vi "ALL - FuncVIs Collection.vi"() -> ()   [LabVIEW 2021]
doc: "::: CalcExpress Toolkit :::\nCopyright (c) 2000-2026 Konstantin Shifershteyn. All rights reserved."
uses:
  cetypes.llb/CalcExpress Instance RefNum.ctl
panel:
  in  "False":bool
  in  "InstanceRef":T1
  # "CalcExpress Toolkit\n\nFuncVI Collection"
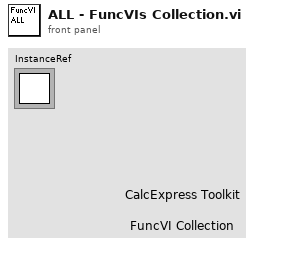
[diagram p1: front panel]
types:
  T1 = typedef "CalcExpress Instance RefNum.ctl" = refnum<k1>
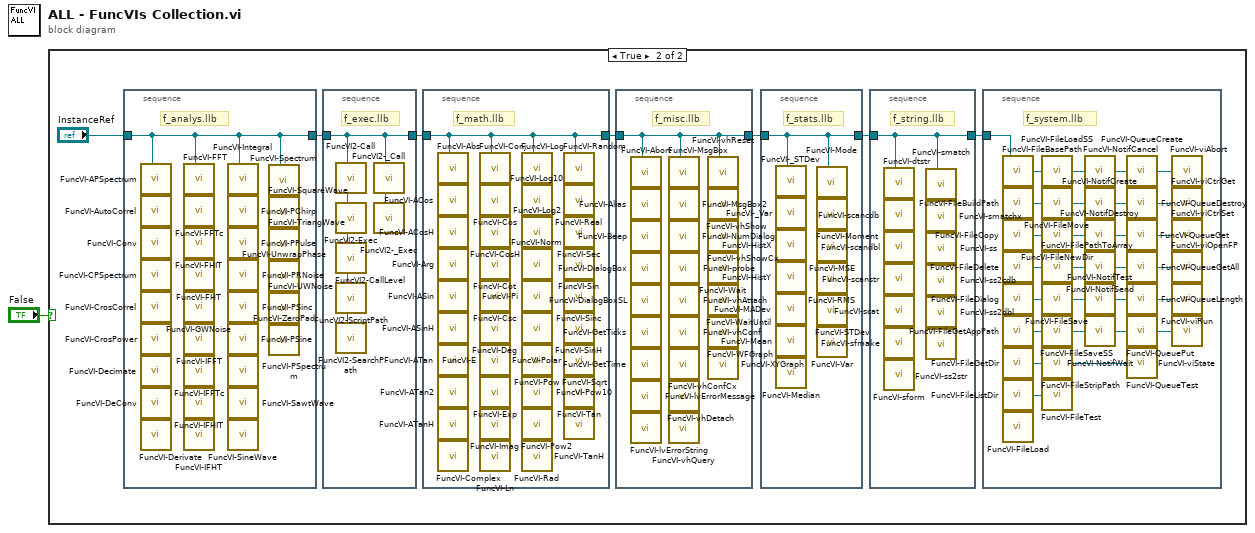
[diagram p0: block diagram]
diagram:
  n1 = case shown="True" "False" {
    frame False {
    }
    frame True {
      n2 = stacked-sequence {
        tunnel: "InstanceRef" -> [w15]
        tunnel: [w15] -> w7
        frame #0 {
          # "f_analys.llb"
          n3 = call "FuncVI-APSpectrum.vi"("InstanceRef"=w15) -> ()  [unwired: 7 in, 2 out]
          n4 = call "FuncVI-AutoCorrel.vi"("InstanceRef"=w15) -> ()  [unwired: 7 in, 2 out]
          n5 = call "FuncVI-Conv.vi"("InstanceRef"=w15) -> ()  [unwired: 7 in, 2 out]
          n6 = call "FuncVI-CPSpectrum.vi"("InstanceRef"=w15) -> ()  [unwired: 7 in, 2 out]
          n7 = call "FuncVI-CrosCorrel.vi"("InstanceRef"=w15) -> ()  [unwired: 7 in, 2 out]
          n8 = call "FuncVI-CrosPower.vi"("InstanceRef"=w15) -> ()  [unwired: 7 in, 2 out]
          n9 = call "FuncVI-Decimate.vi"("InstanceRef"=w15) -> ()  [unwired: 7 in, 2 out]
          n10 = call "FuncVI-DeConv.vi"("InstanceRef"=w15) -> ()  [unwired: 7 in, 2 out]
          n11 = call "FuncVI-Derivate.vi"("InstanceRef"=w15) -> ()  [unwired: 7 in, 2 out]
          n12 = call "FuncVI-FFT.vi"("InstanceRef"=w15) -> ()  [unwired: 7 in, 2 out]
          n13 = call "FuncVI-FFTc.vi"("InstanceRef"=w15) -> ()  [unwired: 7 in, 2 out]
          n14 = call "FuncVI-FHIT.vi"("InstanceRef"=w15) -> ()  [unwired: 7 in, 2 out]
          n15 = call "FuncVI-FHT.vi"("InstanceRef"=w15) -> ()  [unwired: 7 in, 2 out]
          n16 = call "FuncVI-GWNoise.vi"("InstanceRef"=w15) -> ()  [unwired: 7 in, 2 out]
          n17 = call "FuncVI-IFFT.vi"("InstanceRef"=w15) -> ()  [unwired: 7 in, 2 out]
          n18 = call "FuncVI-IFFTc.vi"("InstanceRef"=w15) -> ()  [unwired: 7 in, 2 out]
          n19 = call "FuncVI-IFHIT.vi"("InstanceRef"=w15) -> ()  [unwired: 7 in, 2 out]
          n20 = call "FuncVI-IFHT.vi"("InstanceRef"=w15) -> ()  [unwired: 7 in, 2 out]
          n21 = call "FuncVI-Integral.vi"("InstanceRef"=w15) -> ()  [unwired: 7 in, 2 out]
          n22 = call "FuncVI-PChirp.vi"("InstanceRef"=w15) -> ()  [unwired: 7 in, 2 out]
          n23 = call "FuncVI-PPulse.vi"("InstanceRef"=w15) -> ()  [unwired: 7 in, 2 out]
          n24 = call "FuncVI-PRNoise.vi"("InstanceRef"=w15) -> ()  [unwired: 7 in, 2 out]
          n25 = call "FuncVI-PSinc.vi"("InstanceRef"=w15) -> ()  [unwired: 7 in, 2 out]
          n26 = call "FuncVI-PSine.vi"("InstanceRef"=w15) -> ()  [unwired: 7 in, 2 out]
          n27 = call "FuncVI-PSpectrum.vi"("InstanceRef"=w15) -> ()  [unwired: 7 in, 2 out]
          n28 = call "FuncVI-SawtWave.vi"("InstanceRef"=w15) -> ()  [unwired: 7 in, 2 out]
          n29 = call "FuncVI-SineWave.vi"("InstanceRef"=w15) -> ()  [unwired: 7 in, 2 out]
          n30 = call "FuncVI-Spectrum.vi"("InstanceRef"=w15) -> ()  [unwired: 7 in, 2 out]
          n31 = call "FuncVI-SquareWave.vi"("InstanceRef"=w15) -> ()  [unwired: 7 in, 2 out]
          n32 = call "FuncVI-TriangWave.vi"("InstanceRef"=w15) -> ()  [unwired: 7 in, 2 out]
          n33 = call "FuncVI-UnwrapPhase.vi"("InstanceRef"=w15) -> ()  [unwired: 7 in, 2 out]
          n34 = call "FuncVI-UWNoise.vi"("InstanceRef"=w15) -> ()  [unwired: 7 in, 2 out]
          n35 = call "FuncVI-ZeroPad.vi"("InstanceRef"=w15) -> ()  [unwired: 7 in, 2 out]
        }
      }
      n36 = stacked-sequence {
        tunnel: w7 -> [w14]
        tunnel: [w14] -> w2
        frame #0 {
          # "f_exec.llb"
          n37 = call "FuncVI2-Call.vi"("InstanceRef"=w14) -> ()  [unwired: 7 in, 2 out]
          n38 = call "FuncVI2-Exec.vi"("InstanceRef"=w14) -> ()  [unwired: 7 in, 2 out]
          n39 = call "FuncVI2-CallLevel.vi"("InstanceRef"=w14) -> ()  [unwired: 7 in, 2 out]
          n40 = call "FuncVI2-ScriptPath.vi"("InstanceRef"=w14) -> ()  [unwired: 7 in, 2 out]
          n41 = call "FuncVI2-SearchPath.vi"("InstanceRef"=w14) -> ()  [unwired: 7 in, 2 out]
          n42 = call "FuncVI2-_Call.vi"("InstanceRef"=w14) -> ()  [unwired: 7 in, 2 out]
          n43 = call "FuncVI2-_Exec.vi"("InstanceRef"=w14) -> ()  [unwired: 7 in, 2 out]
        }
      }
      n44 = stacked-sequence {
        tunnel: [w11] -> w3
        tunnel: w2 -> [w11]
        frame #0 {
          # "f_math.llb"
          n45 = call "FuncVI-Abs.vi"("InstanceRef"=w11) -> ()  [unwired: 7 in, 2 out]
          n46 = call "FuncVI-ACos.vi"("InstanceRef"=w11) -> ()  [unwired: 7 in, 2 out]
          n47 = call "FuncVI-ACosH.vi"("InstanceRef"=w11) -> ()  [unwired: 7 in, 2 out]
          n48 = call "FuncVI-Arg.vi"("InstanceRef"=w11) -> ()  [unwired: 7 in, 2 out]
          n49 = call "FuncVI-ASin.vi"("InstanceRef"=w11) -> ()  [unwired: 7 in, 2 out]
          n50 = call "FuncVI-ASinH.vi"("InstanceRef"=w11) -> ()  [unwired: 7 in, 2 out]
          n51 = call "FuncVI-ATan.vi"("InstanceRef"=w11) -> ()  [unwired: 7 in, 2 out]
          n52 = call "FuncVI-ATan2.vi"("InstanceRef"=w11) -> ()  [unwired: 7 in, 2 out]
          n53 = call "FuncVI-ATanH.vi"("InstanceRef"=w11) -> ()  [unwired: 7 in, 2 out]
          n54 = call "FuncVI-Complex.vi"("InstanceRef"=w11) -> ()  [unwired: 7 in, 2 out]
          n55 = call "FuncVI-Conj.vi"("InstanceRef"=w11) -> ()  [unwired: 7 in, 2 out]
          n56 = call "FuncVI-Cos.vi"("InstanceRef"=w11) -> ()  [unwired: 7 in, 2 out]
          n57 = call "FuncVI-CosH.vi"("InstanceRef"=w11) -> ()  [unwired: 7 in, 2 out]
          n58 = call "FuncVI-Cot.vi"("InstanceRef"=w11) -> ()  [unwired: 7 in, 2 out]
          n59 = call "FuncVI-Csc.vi"("InstanceRef"=w11) -> ()  [unwired: 7 in, 2 out]
          n60 = call "FuncVI-Deg.vi"("InstanceRef"=w11) -> ()  [unwired: 7 in, 2 out]
          n61 = call "FuncVI-E.vi"("InstanceRef"=w11) -> ()  [unwired: 7 in, 2 out]
          n62 = call "FuncVI-Exp.vi"("InstanceRef"=w11) -> ()  [unwired: 7 in, 2 out]
          n63 = call "FuncVI-Imag.vi"("InstanceRef"=w11) -> ()  [unwired: 7 in, 2 out]
          n64 = call "FuncVI-Ln.vi"("InstanceRef"=w11) -> ()  [unwired: 7 in, 2 out]
          n65 = call "FuncVI-Log.vi"("InstanceRef"=w11) -> ()  [unwired: 7 in, 2 out]
          n66 = call "FuncVI-Log10.vi"("InstanceRef"=w11) -> ()  [unwired: 7 in, 2 out]
          n67 = call "FuncVI-Log2.vi"("InstanceRef"=w11) -> ()  [unwired: 7 in, 2 out]
          n68 = call "FuncVI-Norm.vi"("InstanceRef"=w11) -> ()  [unwired: 7 in, 2 out]
          n69 = call "FuncVI-Pi.vi"("InstanceRef"=w11) -> ()  [unwired: 7 in, 2 out]
          n70 = call "FuncVI-Polar.vi"("InstanceRef"=w11) -> ()  [unwired: 7 in, 2 out]
          n71 = call "FuncVI-Pow.vi"("InstanceRef"=w11) -> ()  [unwired: 7 in, 2 out]
          n72 = call "FuncVI-Pow10.vi"("InstanceRef"=w11) -> ()  [unwired: 7 in, 2 out]
          n73 = call "FuncVI-Pow2.vi"("InstanceRef"=w11) -> ()  [unwired: 7 in, 2 out]
          n74 = call "FuncVI-Rad.vi"("InstanceRef"=w11) -> ()  [unwired: 7 in, 2 out]
          n75 = call "FuncVI-Random.vi"("InstanceRef"=w11) -> ()  [unwired: 7 in, 2 out]
          n76 = call "FuncVI-Real.vi"("InstanceRef"=w11) -> ()  [unwired: 7 in, 2 out]
          n77 = call "FuncVI-Sec.vi"("InstanceRef"=w11) -> ()  [unwired: 7 in, 2 out]
          n78 = call "FuncVI-Sin.vi"("InstanceRef"=w11) -> ()  [unwired: 7 in, 2 out]
          n79 = call "FuncVI-Sinc.vi"("InstanceRef"=w11) -> ()  [unwired: 7 in, 2 out]
          n80 = call "FuncVI-SinH.vi"("InstanceRef"=w11) -> ()  [unwired: 7 in, 2 out]
          n81 = call "FuncVI-Sqrt.vi"("InstanceRef"=w11) -> ()  [unwired: 7 in, 2 out]
          n82 = call "FuncVI-Tan.vi"("InstanceRef"=w11) -> ()  [unwired: 7 in, 2 out]
          n83 = call "FuncVI-TanH.vi"("InstanceRef"=w11) -> ()  [unwired: 7 in, 2 out]
        }
      }
      n84 = stacked-sequence {
        tunnel: [w10] -> w4
        tunnel: w3 -> [w10]
        frame #0 {
          # "f_misc.llb"
          n85 = call "FuncVI-Abort.vi"("InstanceRef"=w10) -> ()  [unwired: 7 in, 2 out]
          n86 = call "FuncVI-Alias.vi"("InstanceRef"=w10) -> ()  [unwired: 7 in, 2 out]
          n87 = call "FuncVI-Beep.vi"("InstanceRef"=w10) -> ()  [unwired: 7 in, 2 out]
          n88 = call "FuncVI-DialogBox.vi"("InstanceRef"=w10) -> ()  [unwired: 7 in, 2 out]
          n89 = call "FuncVI-DialogBoxSL.vi"("InstanceRef"=w10) -> ()  [unwired: 7 in, 2 out]
          n90 = call "FuncVI-GetTicks.vi"("InstanceRef"=w10) -> ()  [unwired: 7 in, 2 out]
          n91 = call "FuncVI-GetTime.vi"("InstanceRef"=w10) -> ()  [unwired: 7 in, 2 out]
          n92 = call "FuncVI-lvErrorMessage.vi"("InstanceRef"=w10) -> ()  [unwired: 7 in, 2 out]
          n93 = call "FuncVI-lvErrorString.vi"("InstanceRef"=w10) -> ()  [unwired: 7 in, 2 out]
          n94 = call "FuncVI-MsgBox.vi"("InstanceRef"=w10) -> ()  [unwired: 7 in, 2 out]
          n95 = call "FuncVI-MsgBox2.vi"("InstanceRef"=w10) -> ()  [unwired: 7 in, 2 out]
          n96 = call "FuncVI-NumDialog.vi"("InstanceRef"=w10) -> ()  [unwired: 7 in, 2 out]
          n97 = call "FuncVI-probe.vi"("InstanceRef"=w10) -> ()  [unwired: 7 in, 2 out]
          n98 = call "FuncVI-vhAttach.vi"("InstanceRef"=w10) -> ()  [unwired: 7 in, 2 out]
          n99 = call "FuncVI-vhConf.vi"("InstanceRef"=w10) -> ()  [unwired: 7 in, 2 out]
          n100 = call "FuncVI-vhConfCx.vi"("InstanceRef"=w10) -> ()  [unwired: 7 in, 2 out]
          n101 = call "FuncVI-vhDetach.vi"("InstanceRef"=w10) -> ()  [unwired: 7 in, 2 out]
          n102 = call "FuncVI-vhQuery.vi"("InstanceRef"=w10) -> ()  [unwired: 7 in, 2 out]
          n103 = call "FuncVI-vhReset.vi"("InstanceRef"=w10) -> ()  [unwired: 7 in, 2 out]
          n104 = call "FuncVI-vhShow.vi"("InstanceRef"=w10) -> ()  [unwired: 7 in, 2 out]
          n105 = call "FuncVI-vhShowCx.vi"("InstanceRef"=w10) -> ()  [unwired: 7 in, 2 out]
          n106 = call "FuncVI-Wait.vi"("InstanceRef"=w10) -> ()  [unwired: 7 in, 2 out]
          n107 = call "FuncVI-WaitUntil.vi"("InstanceRef"=w10) -> ()  [unwired: 7 in, 2 out]
          n108 = call "FuncVI-WFGraph.vi"("InstanceRef"=w10) -> ()  [unwired: 7 in, 2 out]
          n109 = call "FuncVI-XYGraph.vi"("InstanceRef"=w10) -> ()  [unwired: 7 in, 2 out]
        }
      }
      n110 = stacked-sequence {
        tunnel: [w13] -> w5
        tunnel: w4 -> [w13]
        frame #0 {
          # "f_stats.llb"
          n111 = call "FuncVI-_STDev.vi"("InstanceRef"=w13) -> ()  [unwired: 7 in, 2 out]
          n112 = call "FuncVI-_Var.vi"("InstanceRef"=w13) -> ()  [unwired: 7 in, 2 out]
          n113 = call "FuncVI-HistX.vi"("InstanceRef"=w13) -> ()  [unwired: 7 in, 2 out]
          n114 = call "FuncVI-HistY.vi"("InstanceRef"=w13) -> ()  [unwired: 7 in, 2 out]
          n115 = call "FuncVI-MADev.vi"("InstanceRef"=w13) -> ()  [unwired: 7 in, 2 out]
          n116 = call "FuncVI-Mean.vi"("InstanceRef"=w13) -> ()  [unwired: 7 in, 2 out]
          n117 = call "FuncVI-Median.vi"("InstanceRef"=w13) -> ()  [unwired: 7 in, 2 out]
          n118 = call "FuncVI-Mode.vi"("InstanceRef"=w13) -> ()  [unwired: 7 in, 2 out]
          n119 = call "FuncVI-Moment.vi"("InstanceRef"=w13) -> ()  [unwired: 7 in, 2 out]
          n120 = call "FuncVI-MSE.vi"("InstanceRef"=w13) -> ()  [unwired: 7 in, 2 out]
          n121 = call "FuncVI-RMS.vi"("InstanceRef"=w13) -> ()  [unwired: 7 in, 2 out]
          n122 = call "FuncVI-STDev.vi"("InstanceRef"=w13) -> ()  [unwired: 7 in, 2 out]
          n123 = call "FuncVI-Var.vi"("InstanceRef"=w13) -> ()  [unwired: 7 in, 2 out]
        }
      }
      n124 = stacked-sequence {
        tunnel: [w12] -> w6
        tunnel: w5 -> [w12]
        frame #0 {
          # "f_string.llb"
          n125 = call "FuncVI-dtstr.vi"("InstanceRef"=w12) -> ()  [unwired: 7 in, 2 out]
          n126 = call "FuncVI-scancdb.vi"("InstanceRef"=w12) -> ()  [unwired: 7 in, 2 out]
          n127 = call "FuncVI-scandbl.vi"("InstanceRef"=w12) -> ()  [unwired: 7 in, 2 out]
          n128 = call "FuncVI-scanstr.vi"("InstanceRef"=w12) -> ()  [unwired: 7 in, 2 out]
          n129 = call "FuncVI-scat.vi"("InstanceRef"=w12) -> ()  [unwired: 7 in, 2 out]
          n130 = call "FuncVI-sfmake.vi"("InstanceRef"=w12) -> ()  [unwired: 7 in, 2 out]
          n131 = call "FuncVI-sform.vi"("InstanceRef"=w12) -> ()  [unwired: 7 in, 2 out]
          n132 = call "FuncVI-smatch.vi"("InstanceRef"=w12) -> ()  [unwired: 7 in, 2 out]
          n133 = call "FuncVI-smatchx.vi"("InstanceRef"=w12) -> ()  [unwired: 7 in, 2 out]
          n134 = call "FuncVI-ss.vi"("InstanceRef"=w12) -> ()  [unwired: 7 in, 2 out]
          n135 = call "FuncVI-ss2cdb.vi"("InstanceRef"=w12) -> ()  [unwired: 7 in, 2 out]
          n136 = call "FuncVI-ss2dbl.vi"("InstanceRef"=w12) -> ()  [unwired: 7 in, 2 out]
          n137 = call "FuncVI-ss2str.vi"("InstanceRef"=w12) -> ()  [unwired: 7 in, 2 out]
        }
      }
      n138 = stacked-sequence {
        tunnel: w6 -> [w9]
        frame #0 {
          # "f_system.llb"
          n139 = call "FuncVI-FileBasePath.vi"("InstanceRef"=w9) -> ()  [unwired: 7 in, 2 out]
          n140 = call "FuncVI-FileBuildPath.vi"("InstanceRef"=w9) -> ()  [unwired: 7 in, 2 out]
          n141 = call "FuncVI-FileCopy.vi"("InstanceRef"=w9) -> ()  [unwired: 7 in, 2 out]
          n142 = call "FuncVI-FileDelete.vi"("InstanceRef"=w9) -> ()  [unwired: 7 in, 2 out]
          n143 = call "FuncVI-FileDialog.vi"("InstanceRef"=w9) -> ()  [unwired: 7 in, 2 out]
          n144 = call "FuncVI-FileGetAppPath.vi"("InstanceRef"=w9) -> ()  [unwired: 7 in, 2 out]
          n145 = call "FuncVI-FileGetDir.vi"("InstanceRef"=w9) -> ()  [unwired: 7 in, 2 out]
          n146 = call "FuncVI-FileListDir.vi"("InstanceRef"=w9) -> ()  [unwired: 7 in, 2 out]
          n147 = call "FuncVI-FileLoad.vi"("InstanceRef"=w9) -> ()  [unwired: 7 in, 2 out]
          n148 = call "FuncVI-FileLoadSS.vi"("InstanceRef"=w9) -> ()  [unwired: 7 in, 2 out]
          n149 = call "FuncVI-FileMove.vi"("InstanceRef"=w9) -> ()  [unwired: 7 in, 2 out]
          n150 = call "FuncVI-FileNewDir.vi"("InstanceRef"=w9) -> ()  [unwired: 7 in, 2 out]
          n151 = call "FuncVI-FilePathToArray.vi"("InstanceRef"=w9) -> ()  [unwired: 7 in, 2 out]
          n152 = call "FuncVI-FileSave.vi"("InstanceRef"=w9) -> ()  [unwired: 7 in, 2 out]
          n153 = call "FuncVI-FileSaveSS.vi"("InstanceRef"=w9) -> ()  [unwired: 7 in, 2 out]
          n154 = call "FuncVI-FileStripPath.vi"("InstanceRef"=w9) -> ()  [unwired: 7 in, 2 out]
          n155 = call "FuncVI-FileTest.vi"("InstanceRef"=w9) -> ()  [unwired: 7 in, 2 out]
          n156 = call "FuncVI-NotifCancel.vi"("InstanceRef"=w9) -> ()  [unwired: 7 in, 2 out]
          n157 = call "FuncVI-NotifCreate.vi"("InstanceRef"=w9) -> ()  [unwired: 7 in, 2 out]
          n158 = call "FuncVI-NotifDestroy.vi"("InstanceRef"=w9) -> ()  [unwired: 7 in, 2 out]
          n159 = call "FuncVI-NotifSend.vi"("InstanceRef"=w9) -> ()  [unwired: 7 in, 2 out]
          n160 = call "FuncVI-NotifTest.vi"("InstanceRef"=w9) -> ()  [unwired: 7 in, 2 out]
          n161 = call "FuncVI-NotifWait.vi"("InstanceRef"=w9) -> ()  [unwired: 7 in, 2 out]
          n162 = call "FuncVI-QueueCreate.vi"("InstanceRef"=w9) -> ()  [unwired: 7 in, 2 out]
          n163 = call "FuncVI-QueueDestroy.vi"("InstanceRef"=w9) -> ()  [unwired: 7 in, 2 out]
          n164 = call "FuncVI-QueueGet.vi"("InstanceRef"=w9) -> ()  [unwired: 7 in, 2 out]
          n165 = call "FuncVI-QueueGetAll.vi"("InstanceRef"=w9) -> ()  [unwired: 7 in, 2 out]
          n166 = call "FuncVI-QueueLength.vi"("InstanceRef"=w9) -> ()  [unwired: 7 in, 2 out]
          n167 = call "FuncVI-QueuePut.vi"("InstanceRef"=w9) -> ()  [unwired: 7 in, 2 out]
          n168 = call "FuncVI-QueueTest.vi"("InstanceRef"=w9) -> ()  [unwired: 7 in, 2 out]
          n169 = call "FuncVI-viAbort.vi"("InstanceRef"=w9) -> ()  [unwired: 7 in, 2 out]
          n170 = call "FuncVI-viCtrlGet.vi"("InstanceRef"=w9) -> ()  [unwired: 7 in, 2 out]
          n171 = call "FuncVI-viCtrlSet.vi"("InstanceRef"=w9) -> ()  [unwired: 7 in, 2 out]
          n172 = call "FuncVI-viOpenFP.vi"("InstanceRef"=w9) -> ()  [unwired: 7 in, 2 out]
          n173 = call "FuncVI-viRun.vi"("InstanceRef"=w9) -> ()  [unwired: 7 in, 2 out]
          n174 = call "FuncVI-viState.vi"("InstanceRef"=w9) -> ()  [unwired: 7 in, 2 out]
        }
      }
    }
  }
